vi "RemoteVI Other Shares.vi"(0 "port":u16=8088) -> (4 "hWnds":u64[](array[numeric]))   [LabVIEW 2020, in "RemoteVI.lvlib"]
doc: "The windows the OTHER running shares of this LabVIEW application instance publish (every share but the one on port; RemoteVI Status Registry.vi, running = published within 2 s). RemoteVI Track Windows.vi does not list them as windows of this share: two VIs shared from one LabVIEW are both running front panels, and each would otherwise show the other's panel as one of its own windows."
uses:
  RemoteVI.lvlib
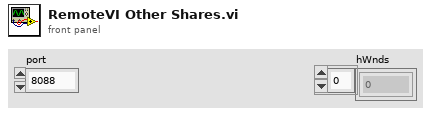
[diagram p1: front panel]
types:
  T1 = cluster{"port":u16, "url":string, "target":string, "kind":string, "whole network":bool, "started":dbl, "updated":dbl, "clients":cluster{"address":string, "since":dbl, "last input":dbl}[], "fps":dbl, "bytes per s":dbl, "frames":u32, "latency ms":dbl, "view only":bool, "last error":string, "hWnd":u64}[]
  T2 = cluster{"port":u16, "url":string, "target":string, "kind":string, "whole network":bool, "running":bool, "uptime s":dbl, "clients":cluster{"address":string, "connected s":dbl, "idle s":dbl}[], "fps":dbl, "kB per s":dbl, "frames":u32, "latency ms":dbl, "view only":bool, "last error":string, "hWnd":u64}[]
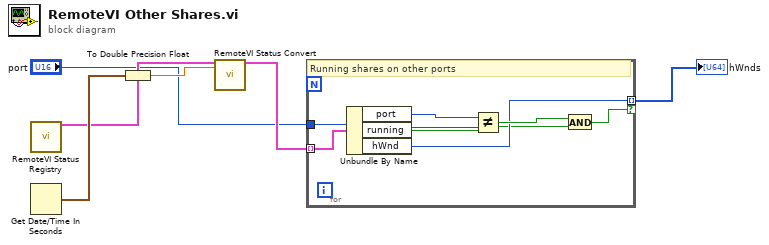
[diagram p0: block diagram]
diagram:
  n1 = call "RemoteVI Status Registry.vi"() -> ("servers"=w2:T1)  [unwired: 15 in]
  n2 = Get Date/Time In Seconds() -> (seconds since 1Jan1904=w3:timestamp)
  n3 = To Double Precision Float(number=w3) -> (double precision float=w4:dbl)
  n4 = call "RemoteVI Status Convert.vi"("raw"=w2, "now"=w4) -> ("status"=w5:T2)  [unwired: 13 in]
  n5 = for {
    tunnel: "port" -> [w8]
    tunnel: w5 -> [w7] mode=indexing
    tunnel: [w11] -> w6 mode=indexing if=w13
    # "Running shares on other ports"
    n6 = Unbundle By Name(w7) -> ("port"=w9:u16, "running"=w10:bool, "hWnd"=w11:u64)
    n7 = Not Equal?(x=w9, y=w8) -> (x != y?=w12:bool)
    n8 = And(x=w12, y=w10) -> (x .and. y?=w13:bool)
  }
  "hWnds" <- w6
